vi "Fire_Stop_Event.vi"(8 "error in (no error)":errorcluster={"status"=FALSE, "code"=0, "source"="\"\""}, 11 "User Event - Stop":refnum<user-event>) -> (0 "error out":errorcluster)   [LabVIEW 2026]
doc: "Send the Stop event to stop parallel loops."
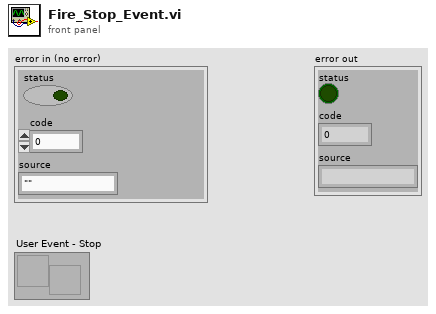
[diagram p1: front panel]
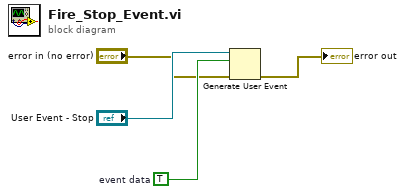
[diagram p0: block diagram]
diagram:
  w3 = TRUE  # event data
  n1 = Generate User Event(user event="User Event - Stop", event data cluster=w3, error in="error in (no error)") -> (error out=→"error out":errorcluster)  [unwired: 1 in, 1 out]
